vi "FuncVI-Spectrum.vi"(5 "InstanceRef":T2, 9 "arg list":T1[](array[typedef]) {"num" format="%.2f"}) -> (0 "error out":bool, 3 "result":T1 {"num" format="%.2f"})   [LabVIEW 2021]
doc: "::: CalcExpress Toolkit :::\nCopyright (c) 2000-2026 Konstantin Shifershteyn. All rights reserved."
uses:
  cetypes.llb/CalcExpress Function Argument Info.ctl
  cetypes.llb/CalcExpress Instance RefNum.ctl
  <vilib>/Analysis/NI_AALPro.lvlib
panel:
  in  "max arg num":i32=5
  in  "min arg num":i32=2
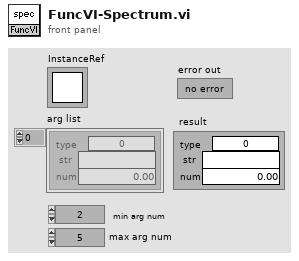
[diagram p1: front panel]
types:
  T1 = typedef "CalcExpress Function Argument Info.ctl" = cluster{"type":u32, "str":string, "num":dbl}
  T2 = typedef "CalcExpress Instance RefNum.ctl" = refnum<k1>
  T3 = enum8{"String", "DBL Number", "identifier", "1D Array of DBL", "2D Array of DBL", "CDB Number", "1D Array of CDB", "2D Array of CDB", "1D Array of String", "2D Array of String", "Unknown data type"}
  T4 = cluster{"index":i32, "type":enum8{"String", "DBL Number", "identifier", "1D Array of DBL", "2D Array of DBL", "CDB Number", "1D Array of CDB", "2D Array of CDB", "Unknown data type"}, "default num":dbl, "default str":string}[]
  T5 = cluster{"num list[0]":dbl, "num list[1]":dbl, "num list[2]":dbl, "num list[3]":dbl, "num list[4]":dbl}
  T6 = typedef "VarMan Variable Context Handle.ctl" = i32
  T7 = cluster{"type":enum8{"String", "DBL Number", "identifier", "1D Array of DBL", "2D Array of DBL", "CDB Number", "1D Array of CDB", "2D Array of CDB", "1D Array of String", "2D Array of String", "Unknown data type"}, string, "df":dbl}
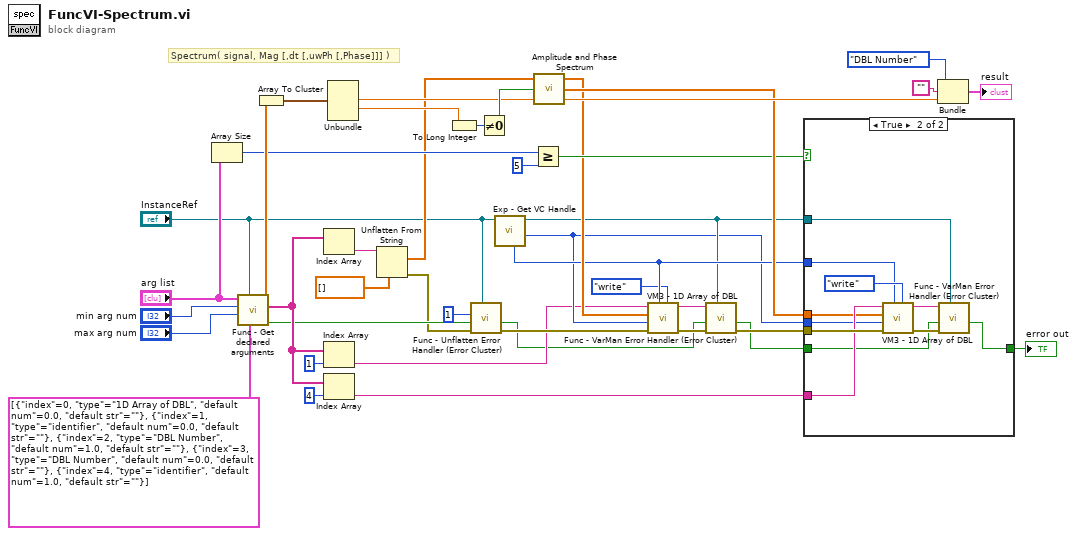
[diagram p0: block diagram]
diagram:
  # "Spectrum( signal, Mag [,dt [,uwPh [,Phase]]] )"
  n1 = Array Size(array="arg list") -> (size(s)=w33:i32)
  n2 = call "Func - Get declared arguments.vi"("arg descriptors"=T4 [{"index"=0, "type"=enum."1D Array of DBL", "default num"=0.0, "default str"=""}, {"index"=1, "type"=enum."identifier", "default num"=0.0, "default str"=""}, {"index"=2, "type"=enum."DBL Number", "default num"=1.0, "default str"=""}, {"index"=3, "type"=enum."DBL Number", "default num"=0.0, "default str"=""}, {"index"=4, "type"=enum."identifier", "default num"=1.0, "default str"=""}] ("args descriptors"), "InstanceRef"="InstanceRef", "max arg num"="max arg num", "min arg num"="min arg num", "arg list"="arg list") -> ("error out"=w15:bool, "str list"=w28:string[], "num list"=w40:dbl[])  [unwired: 3 in, 1 out]
  n3 = Array To Cluster(array=w40) -> (cluster=w39:T5)
  n4 = Index Array(array=w28) -> (element=w23:string)  [unwired: 1 in]
  n5 = Index Array(array=w28, index=1) -> (element=w3:string)
  n6 = Index Array(array=w28, index=4) -> (element=w19:string)
  n7 = Unbundle(w39) -> ("num list[2]"=w26:dbl, "num list[3]"=w25:dbl)  [unwired: 3 out]
  n8 = Unflatten From String(type=dbl[] [] ("value out"), binary string=w23) -> (value=w21:dbl[], error out=w14:errorcluster)  [unwired: 3 in, 1 out]
  n9 = To Long Integer(number=w25) -> (32bit integer=w37:i32)
  n10 = call "Func - Unflatten Error Handler (Error Cluster).vi"("InstanceRef"="InstanceRef", "Unflatten Error Cluster"=w14, "error status before"=w15, "argument number"=1) -> ("Error Cluster out"=w12:errorcluster, "error status out"=w1:bool)  [unwired: 5 in, 1 out]
  n11 = Not Equal To 0?(x=w37) -> (x != 0?=w32:bool)
  n12 = call "Exp - Get VC Handle.vi"("InstanceRef"="InstanceRef") -> ("writer ID"=w4:u32, "dup InstanceRef"=w6:T2, "VC Handle"=w10:T6)  [unwired: 5 in, 1 out]
  n13 = Greater Or Equal?(x=w33, y=5) -> (x >= y?=w35:bool)
  n14 = call <vilib>:"Amplitude and Phase Spectrum.vi"("dt"=w26, "unwrap phase (T)"=w32, "Signal (V)"=w21) -> ("df"=w38:dbl, "Amp Spectrum Phase (radians)"=w36:dbl[], "Amp Spectrum Mag (Vrms)"=w11:dbl[])
  n15 = call "VM3 - 1D Array of DBL.vi"("cmd (read)"=enum16{"create", "destroy", "write", "read"}."write", "VC Handle"=w10, "error in"=w12, "writer ID"=w4, "value in"=w11, "name_spec"=w3) -> ("error out"=w8:errorcluster, "dup name_spec"=w7:string)  [unwired: 2 in, 2 out]
  n16 = call "Func - VarMan Error Handler (Error Cluster).vi"("InstanceRef"=w6, "VarMan VI error in"=w8, "error status before"=w1, "var name"=w7) -> ("error out"=w5:errorcluster, "FuncVI error out"=w2:bool)  [unwired: 5 in, 1 out]
  n17 = case shown="True" w35 {
    tunnel: w36 -> [_ w49]
    tunnel: [w43 w45] -> w20
    tunnel: w6 -> [_ w47]
    tunnel: w10 -> [_ w46]
    tunnel: w19 -> [_ w50]
    tunnel: w5 -> [_ w51]
    tunnel: w4 -> [_ w48]
    tunnel: w2 -> [w43 w44]
    frame False {
    }
    frame True {
      n18 = call "VM3 - 1D Array of DBL.vi"("cmd (read)"=enum16{"create", "destroy", "write", "read"}."write", "VC Handle"=w46, "error in"=w51, "writer ID"=w48, "value in"=w49, "name_spec"=w50) -> ("error out"=w53:errorcluster, "dup name_spec"=w54:string)  [unwired: 2 in, 2 out]
      n19 = call "Func - VarMan Error Handler (Error Cluster).vi"("InstanceRef"=w47, "VarMan VI error in"=w53, "error status before"=w44, "var name"=w54) -> ("FuncVI error out"=w45:bool)  [unwired: 5 in, 2 out]
    }
  }
  "error out" <- w20
  n20 = Bundle("type"=T3."DBL Number", "", "df"=w38) -> (→"result":T7)  [unwired: 1 in]
